vi "RemoteVI Check WS Decode Client Frame.vi"() -> (4 "labels":string[](array[string]), 6 "expected":string[](array[string]), 8 "actual":string[](array[string]), 10 "failures":i32)   [LabVIEW 2020]
doc: "Test support, generated by tests/caraya/build.py from tests/vectors/websocket.json (clientFrames, incompleteClientFrames) - do not edit. Calls RemoteVI WS Decode Client Frame.vi once per vector: a valid frame must decode completely with its fin, opcode and payload, bytes consumed = the frame length (as the JS tests assert) and close code 0; an invalid frame must give complete? FALSE and the vector's close code; an incomplete prefix complete? FALSE and close code 0. max payload keeps its default (65536, the JS limit). Outputs, one element per vector: labels (the vector's name), expected (rendered from the vector), actual (the VI's result rendered the same way), and failures, the number of vectors whose expected and actual differ."
uses:
  source/RemoteVI.lvlib
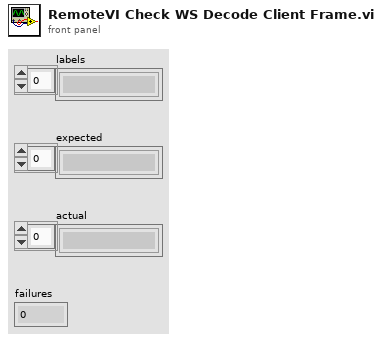
[diagram p1: front panel]
types:
  T1 = cluster{"name":string, "frame":string, "full":bool, "expect":string}[]
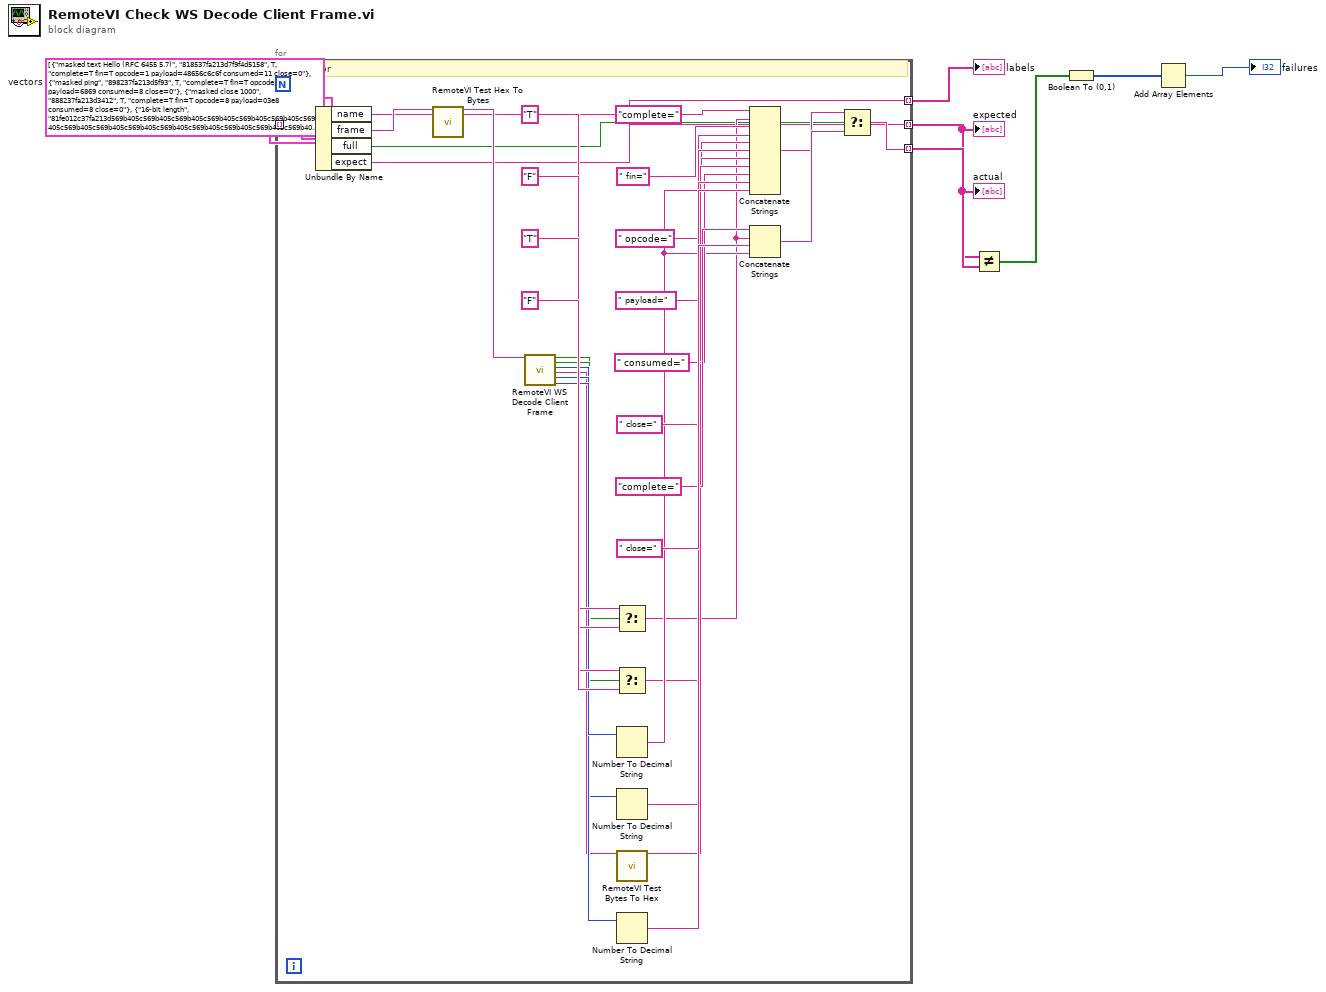
[diagram p0: block diagram]
diagram:
  w1 = T1 [{"name"="masked text Hello (RFC 6455 5.7)", "frame"="818537fa213d7f9f4d5158", "full"=TRUE, "expect"="complete=T fin=T opcode=1 payload=48656c6c6f consumed=11 close=0"}, {"name"="masked ping", "frame"="898237fa213d5f93", "full"=TRUE, "expect"="complete=T fin=T opcode=9 payload=6869 consumed=8 close=0"}, {"name"="masked close 1000", "frame"="888237fa213d3412", "full"=TRUE, "expect"="complete=T fin=T opcode=8 payload=03e8 consumed=8 close=0"}, {"name"="16-bit length", "frame"="81fe012c37fa213d569b405c569b405c569b405c569b405c569b405c569b405c569b405c569b405c569b405c569b405c569b405c569b405c569b405c569b405c569b405c569b405c569b405c569b405c569b405c569b405c569b405c569b405c569b405c569b405c569b405c569b405c569b405c569b405c569b405c569b405c569b405c569b405c569b405c569b405c569b405c569b405c569b405c569b405c569b405c569b405c569b405c569b405c569b405c569b405c569b405c569b405c569b405c569b405c569b405c569b405c569b405c569b405c569b405c569b405c569b405c569b405c569b405c569b405c569b405c569b405c569b405c569b405c569b405c569b405c569b405c569b405c569b405c569b405c569b405c569b405c569b405c569b405c569b405c569b405c569b405c", "full"=TRUE, "expect"="complete=T fin=T opcode=1 payload=616161616161616161616161616161616161616161616161616161616161616161616161616161616161616161616161616161616161616161616161616161616161616161616161616161616161616161616161616161616161616161616161616161616161616161616161616161616161616161616161616161616161616161616161616161616161616161616161616161616161616161616161616161616161616161616161616161616161616161616161616161616161616161616161616161616161616161616161616161616161616161616161616161616161616161616161616161616161616161616161616161616161616161616161616161616161616161616161616161616161616161616161616161616161616161616161616161616161616161616161 consumed=308 close=0"}, {"name"="empty text", "frame"="818037fa213d", "full"=TRUE, "expect"="complete=T fin=T opcode=1 payload= consumed=6 close=0"}, {"name"="unmasked (RFC 6455 5.7, client->server forbidden)", "frame"="810548656c6c6f", "full"=FALSE, "expect"="complete=F close=1002"}, {"name"="RSV1 set", "frame"="c18137fa213d4f", "full"=FALSE, "expect"="complete=F close=1002"}, {"name"="reserved opcode 3", "frame"="838137fa213d4f", "full"=FALSE, "expect"="complete=F close=1002"}, {"name"="fragmented ping", "frame"="098137fa213d4f", "full"=FALSE, "expect"="complete=F close=1002"}, {"name"="control frame > 125 bytes", "frame"="89fe007e37fa213d37fa213d37fa213d37fa213d37fa213d37fa213d37fa213d37fa213d37fa213d37fa213d37fa213d37fa213d37fa213d37fa213d37fa213d37fa213d37fa213d37fa213d37fa213d37fa213d37fa213d37fa213d37fa213d37fa213d37fa213d37fa213d37fa213d37fa213d37fa213d37fa213d37fa213d37fa213d37fa", "full"=FALSE, "expect"="complete=F close=1002"}, {"name"="64-bit length beyond limit", "frame"="81ff000000010000000000000000", "full"=FALSE, "expect"="complete=F close=1009"}, {"name"="incomplete prefix ''", "frame"="", "full"=FALSE, "expect"="complete=F close=0"}, {"name"="incomplete prefix '81'", "frame"="81", "full"=FALSE, "expect"="complete=F close=0"}, {"name"="incomplete prefix '81fe'", "frame"="81fe", "full"=FALSE, "expect"="complete=F close=0"}, {"name"="incomplete prefix '81fe01'", "frame"="81fe01", "full"=FALSE, "expect"="complete=F close=0"}, {"name"="incomplete prefix '8185'", "frame"="8185", "full"=FALSE, "expect"="complete=F close=0"}, {"name"="incomplete prefix '818537fa'", "frame"="818537fa", "full"=FALSE, "expect"="complete=F close=0"}, {"name"="incomplete prefix '818537fa213d7f9f4d51'", "frame"="818537fa213d7f9f4d51", "full"=FALSE, "expect"="complete=F close=0"}]  # vectors
  n1 = for {
    tunnel: w1 -> [w8] mode=indexing
    tunnel: [w9] -> w2 mode=indexing
    tunnel: [w12] -> w3 mode=indexing
    tunnel: [w40] -> w4 mode=indexing
    # "One vector"
    n2 = Unbundle By Name(w8) -> ("name"=w9:string, "frame"=w10:string, "full"=w11:bool, "expect"=w12:string)
    n3 = call "RemoteVI Test Hex To Bytes.vi"("hex"=w10) -> ("bytes"=w13:string)  [unwired: 14 in]
    n4 = call "RemoteVI WS Decode Client Frame.vi"("buffer"=w13) -> ("complete?"=w14:bool, "fin"=w15:bool, "opcode"=w16:u8, "payload"=w17:string, "bytes consumed"=w18:u32, "close code"=w19:u16)  [unwired: 13 in]
    n5 = Select(t="T", s=w14, f="F") -> (s? t:f=w22:string)
    n6 = Select(t="T", s=w15, f="F") -> (s? t:f=w25:string)
    n7 = Number To Decimal String(number=w19) -> (decimal integer string=w26:string)  [unwired: 1 in]
    n8 = Number To Decimal String(number=w16) -> (decimal integer string=w30:string)  [unwired: 1 in]
    n9 = call "RemoteVI Test Bytes To Hex.vi"("bytes"=w17) -> ("hex"=w32:string)  [unwired: 14 in]
    n10 = Number To Decimal String(number=w18) -> (decimal integer string=w34:string)  [unwired: 1 in]
    n11 = Concatenate Strings("complete=", w22, " fin=", w25, " opcode=", w30, " payload=", w32, " consumed=", w34, " close=", w26) -> (w36:string)
    n12 = Concatenate Strings("complete=", w22, " close=", w26) -> (w39:string)
    n13 = Select(t=w36, s=w11, f=w39) -> (s? t:f=w40:string)
  }
  "labels" <- w2
  "expected" <- w3
  "actual" <- w4
  n14 = Not Equal?(x=w3, y=w4) -> (x != y?=w5:bool[])
  n15 = Boolean To (0,1)(Boolean=w5) -> (0, 1=w6:i16[])
  n16 = Add Array Elements(numeric array=w6) -> (sum=→"failures":i16)
